vi "LabApp - Get Datalog Directory Path.vi"(10 "Ena Create (F)":bool) -> (2 "created":bool, 3 "path":path)   [LabVIEW 2021]
doc: "::: CalcExpress Toolkit :::\nCopyright (c) 2000-2026 Konstantin Shifershteyn. All rights reserved."
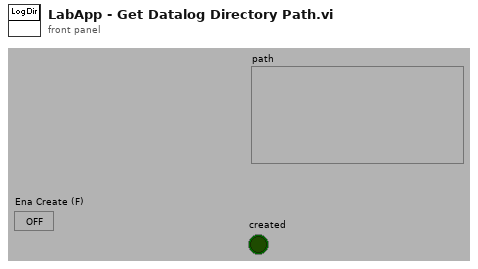
[diagram p1: front panel]
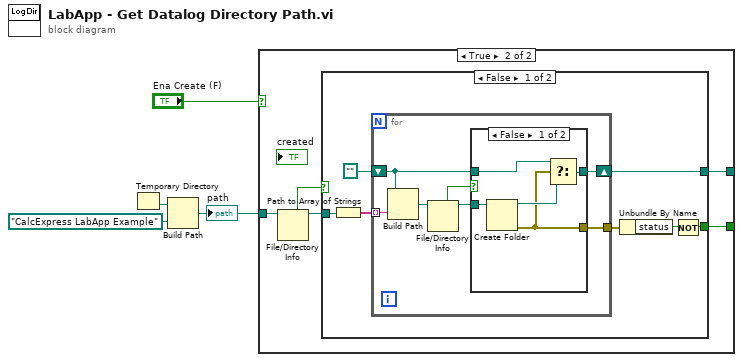
[diagram p0: block diagram]
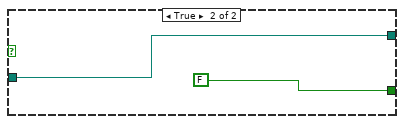
[diagram p4: hidden frame]
diagram:
  n1 = Temporary Directory() -> (w4:path)
  n2 = Build Path(base path=w4, name or relative path=path "CalcExpress LabApp Example") -> (appended path=w1:path)
  "path" <- w1
  n3 = case shown="True" "Ena Create (F)" {
    tunnel: [w5 w8] -> _
    tunnel: [_ w7] -> _
    tunnel: w1 -> [w5 w6]
    frame False {
    }
    frame True {
      n4 = File/Directory Info(path=w6) -> (path out=w9:path, directory=w10:bool)  [unwired: 1 in, 5 out]
      n5 = case shown="False" w10 {
        tunnel: w9 -> [w17 w31]
        tunnel: [w14 w31] -> w8
        tunnel: [w12 FALSE] -> w7
        frame False {
          n6 = Path to Array of Strings(0:w17) -> (2:w16:string[])  [unwired: 1 out]
          n7 = for {
            tunnel: w16 -> [w24] mode=indexing
            shift-right: [w22] -> w14
            shift-left: path "" -> [w19]
            tunnel: [w18] -> w11
            n8 = Build Path(base path=w19, name or relative path=w24) -> (appended path=w21:path)
            n9 = File/Directory Info(path=w21) -> (path out=w20:path, directory=w23:bool)  [unwired: 1 in, 5 out]
            n10 = case shown="False" w23 {
              tunnel: [w28 w30] -> w22
              tunnel: w20 -> [w29 w30]
              tunnel: w19 -> [w26 _]
              tunnel: [w25 _] -> w18
              frame False {
                n11 = Create Folder(path (use dialog)=w29) -> (created path=w27:path, error out=w25:errorcluster)  [unwired: 1 in, 2 out]
                n12 = Select(t=w26, s=w25, f=w27) -> (s? t:f=w28:path)
              }
              frame True {
              }
            }
          }
          n13 = Unbundle By Name(w11) -> ("status"=w13:bool)
          n14 = Not(x=w13) -> (.not. x?=w12:bool)
        }
        frame True {
        }
      }
    }
  }
